vi "Untitled 1.vi"   [LabVIEW 2017]
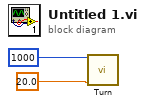
[diagram p0: block diagram]
diagram:
  n1 = call "Turn.vi"("Speed (0-30)"=20.0, "Angle (degrees)"=1000 ("Distance (mm)")) -> ()  [unwired: 10 in]
